vi "Data_Send.vi"(8 "error in (no error)":errorcluster, 10 "rt fifo ref in":refnum<k33>, 11 "Refnum in":refnum<k21>) -> (0 "error out":errorcluster, 3 "Refnum out":refnum<k21>)   [LabVIEW 2025]
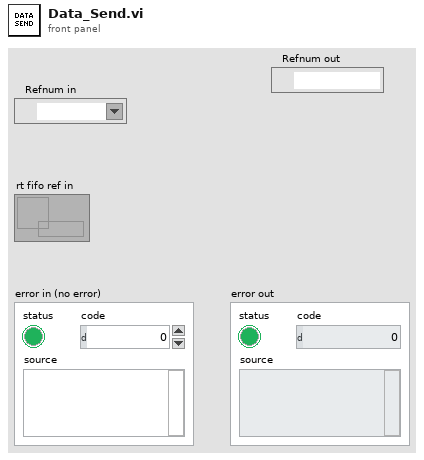
[diagram p1: front panel]
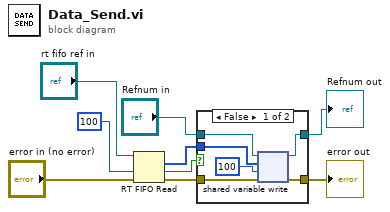
[diagram p0: block diagram]
diagram:
  n1 = RT FIFO Read(0:"rt fifo ref in", 2:100 ("timeout in ms (0)"), 3:"error in (no error)") -> (9:w4:i16[], 10:w3:bool, 11:w7:errorcluster)  [unwired: 1 in, 2 out]
  n2 = case shown="False" w3 {
    tunnel: [w15 w16] -> w1
    tunnel: [w14 w17] -> w9
    tunnel: w4 -> [w12 _]
    tunnel: "Refnum in" -> [w11 w16]
    tunnel: w7 -> [w10 w17]
    frame False {
      n3 = shared-variable-write(w11, w10, w12, 100 ("timeout ms (-1)")) -> (w15:refnum<k21>, w14:errorcluster)  [unwired: 1 out]
    }
    frame True {
    }
  }
  "error out" <- w9
  "Refnum out" <- w1
